vi "Parse Handover Param (L).vi"(8 "error in (no error)":errorcluster caption="에러 입력(에러 없음)", 10 "JSON string":string, 11 "Instrument Manager 입력":refnum<class "Instrument Manager.lvclass">) -> (0 "error out":errorcluster caption="에러 출력", 1 "NR Call Handover Param":T2, 2 "Call Handover Param":T1, 3 "Instrument Manager 출력":refnum<class "Instrument Manager.lvclass">)   [LabVIEW 2023, in "Instrument Manager.lvclass"]
uses:
  Instrument Manager.lvclass
  Type Definition/NR Handover Param.ctl
  Module/ANRITSU Call Box/Type Definition/NR Modulation Type.ctl
  Handover Param.ctl
  Instrument Manager.lvclass/Instrument Manager.ctl
  Module/ANRITSU Call Box/ANRITSU Call Box.lvlib
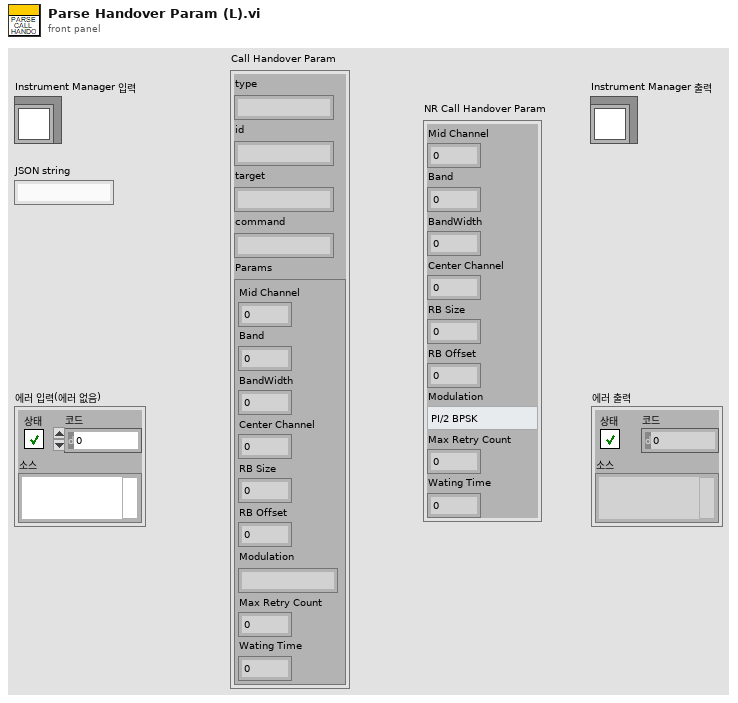
[diagram p1: front panel]
types:
  T1 = typedef "Instrument Manager.lvclass/Handover Param.ctl" = cluster{"type":string, "id":string, "target":string, "command":string, "Params":cluster{"Mid Channel":u32, "Band":u32, "BandWidth":u32, "Center Channel":u32, "RB Size":i32, "RB Offset":i32, "Modulation":string, "Max Retry Count":i32, "Wating Time":i32}}
  T2 = typedef "NR Handover Param.ctl" = cluster{"Mid Channel":u32, "Band":u32, "BandWidth":u32, "Center Channel":u32, "RB Size":i32, "RB Offset":i32, "Modulation":T3, "Max Retry Count":i32, "Wating Time":i32}
  T3 = typedef "ANRITSU Call Box.lvlib/NR Modulation Type.ctl" = enum16{"PI/2 BPSK", "QPSK", "16QAM", "64QAM", "256QAM"}
  T4 = cluster{"Mid Channel":u32, "Band":u32, "BandWidth":u32, "Center Channel":u32, "RB Size":i32, "RB Offset":i32, "Modulation":string, "Max Retry Count":i32, "Wating Time":i32}
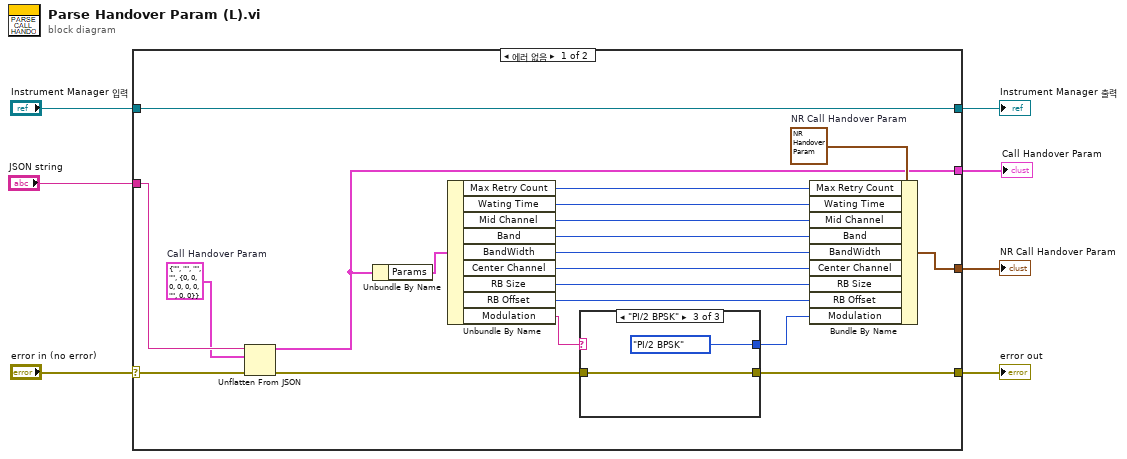
[diagram p0: block diagram]
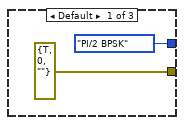
[diagram p2: hidden frame]
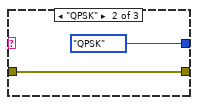
[diagram p3: hidden frame]
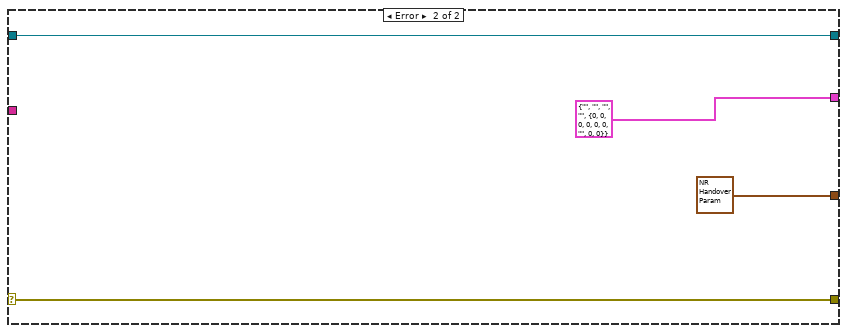
[diagram p4: hidden frame]
diagram:
  n1 = case shown="에러 없음" "error in (no error)" {
    selector: "error in (no error)" -> [w24 w37]
    tunnel: [w10 w37] -> w6
    tunnel: [w27 w36] -> w4
    tunnel: "Instrument Manager 입력" -> [w27 w36]
    tunnel: "JSON string" -> [w26 _]
    tunnel: [w20 T2 {"Mid Channel"=0, "Band"=0, "BandWidth"=0, "Center Channel"=0, "RB Size"=0, "RB Offset"=0, "Modulation"=enum."PI/2 BPSK", "Max Retry Count"=0, "Wating Time"=0} ("NR Call Handover Param")] -> w2
    tunnel: [w19 T1 {"type"="", "id"="", "target"="", "command"="", "Params"={"Mid Channel"=0, "Band"=0, "BandWidth"=0, "Center Channel"=0, "RB Size"=0, "RB Offset"=0, "Modulation"="", "Max Retry Count"=0, "Wating Time"=0}} ("Call Handover Param")] -> w1
    frame No Error {
      w25 = T1 {"type"="", "id"="", "target"="", "command"="", "Params"={"Mid Channel"=0, "Band"=0, "BandWidth"=0, "Center Channel"=0, "RB Size"=0, "RB Offset"=0, "Modulation"="", "Max Retry Count"=0, "Wating Time"=0}}  # Call Handover Param
      w23 = T2 {"Mid Channel"=0, "Band"=0, "BandWidth"=0, "Center Channel"=0, "RB Size"=0, "RB Offset"=0, "Modulation"=enum."PI/2 BPSK", "Max Retry Count"=0, "Wating Time"=0}  # NR Call Handover Param
      n2 = Unflatten From JSON(JSON string=w26, type and defaults=w25, error in (no error)=w24) -> (value=w19:T1, error out=w12:errorcluster)  [unwired: 4 in]
      n3 = Unbundle By Name(w19) -> ("Params"=w22:T4)
      n4 = Unbundle By Name(w22) -> ("Max Retry Count"=w9:i32, "Wating Time"=w8:i32, "Mid Channel"=w18:u32, "Band"=w17:u32, "BandWidth"=w16:u32, "Center Channel"=w15:u32, "RB Size"=w14:i32, "RB Offset"=w13:i32, "Modulation"=w21:string)
      n5 = case shown="\"PI/2 BPSK\"" w21 {
        tunnel: w12 -> [_ w30 w32]
        tunnel: [NR_Modulation_Type."PI/2 BPSK" ("Modulation") NR_Modulation_Type."QPSK" ("Modulation") NR_Modulation_Type."PI/2 BPSK" ("Modulation")] -> w11
        tunnel: [errorcluster {"status"=TRUE, "code"=0, "source"=""} ("error out") w30 w32] -> w10
        frame Default {
        }
        frame "QPSK" {
        }
        frame "PI/2 BPSK" {
        }
      }
      n6 = Bundle By Name(cluster=w23, "Max Retry Count"=w9, "Wating Time"=w8, "Mid Channel"=w18, "Band"=w17, "BandWidth"=w16, "Center Channel"=w15, "RB Size"=w14, "RB Offset"=w13, "Modulation"=w11) -> (w20:T2)
    }
    frame Error {
    }
  }
  "error out" <- w6
  "Instrument Manager 출력" <- w4
  "NR Call Handover Param" <- w2
  "Call Handover Param" <- w1
